vi "SET_ToolGraphic.vi"(8 "error in":errorcluster, 9 "Temp Coord":T5, 10 "Temp Icon":picture, 11 "Data in":T1={"Class"={"Ants"=refnum, "Layer"=refnum, "Templates"=refnum, "Icon"=refnum, "Glyph"=refnum, "Settings"=refnum, "Tools"=refnum, "History"=refnum}, "Ref"={"Add Layer"=refnum, "Remove Layer"=refnum, "Line Text"=[], "Body Text Spec"=refnum, "DNL_Font"=refnum, "glyph path str"=refnum, "templates path str"=refnum, "Arrow Up"=refnum, "Arrow Down"=refnum, "IE VI Ref"=refnum, "Glyphs tree"=refnum, "Templates tree"=refnum, "Layer Icon Text"=refnum, "Layer Template"=refnum, "Body Text"=refnum, "Search Templates"=refnum, "TextMarker"=refnum, "Tab Control"=refnum, "Search Glyphs"=refnum, "Line Color"=refnum, "DNL_Glyphs []"=refnum, "Fill Color"=refnum, "Tools"=refnum, "Icon"=refnum, "Preview"=refnum, "Ants"=refnum, "Terminals"=refnum, "menu reference"=refnum, "LayerNames"=[], "GlyphLoadAnimation"=refnum, "TemplateLoadAnimation"=refnum, "refreshGlyphs"=refnum, "refreshTemplates"=refnum}, "Support"={"AntsRect"={"left"=0, "top"=0, "right"=0, "bottom"=0}, "Mouse Move Coords"={"Horizontal"=0, "Vertical"=0}, "Mouse Down Coords"={"Horizontal"=0, "Vertical"=0}, "Temp Coord"={"Horizontal"=0, "Vertical"=0}, "Action"=enum."Default", "Edge Color"=4914962, "Fill Color"=16860, "Mouse Down?"=FALSE, "Draft Mode?"=FALSE, "Temp Icon"=bytes[3102], "CTRL Pressed"=FALSE, "Move Selection?"=FALSE, "AntsRect Orig"={"left"=0, "top"=0, "right"=0, "bottom"=0}, "Text"="", "TM Set?"=FALSE, "Mouse inside icon?"=FALSE, "Tool (old value)"=0, "Pencil Move Color"=0, "Swap Colors?"=FALSE, "Shift pressed?"=FALSE}}) -> (0 "error out":errorcluster, 1 "All Layers":refnum<class "Layer.lvclass">[](array[class]), 3 "Data out":T1={"Class"={"Ants"=refnum, "Layer"=refnum, "Templates"=refnum, "Icon"=refnum, "Glyph"=refnum, "Settings"=refnum, "Tools"=refnum, "History"=refnum}, "Ref"={"Add Layer"=refnum, "Remove Layer"=refnum, "Line Text"=[], "Body Text Spec"=refnum, "DNL_Font"=refnum, "glyph path str"=refnum, "templates path str"=refnum, "Arrow Up"=refnum, "Arrow Down"=refnum, "IE VI Ref"=refnum, "Glyphs tree"=refnum, "Templates tree"=refnum, "Layer Icon Text"=refnum, "Layer Template"=refnum, "Body Text"=refnum, "Search Templates"=refnum, "TextMarker"=refnum, "Tab Control"=refnum, "Search Glyphs"=refnum, "Line Color"=refnum, "DNL_Glyphs []"=refnum, "Fill Color"=refnum, "Tools"=refnum, "Icon"=refnum, "Preview"=refnum, "Ants"=refnum, "Terminals"=refnum, "menu reference"=refnum, "LayerNames"=[], "GlyphLoadAnimation"=refnum, "TemplateLoadAnimation"=refnum, "refreshGlyphs"=refnum, "refreshTemplates"=refnum}, "Support"={"AntsRect"={"left"=0, "top"=0, "right"=0, "bottom"=0}, "Mouse Move Coords"={"Horizontal"=0, "Vertical"=0}, "Mouse Down Coords"={"Horizontal"=0, "Vertical"=0}, "Temp Coord"={"Horizontal"=0, "Vertical"=0}, "Action"=enum."Default", "Edge Color"=4914962, "Fill Color"=16860, "Mouse Down?"=FALSE, "Draft Mode?"=FALSE, "Temp Icon"=bytes[3102], "CTRL Pressed"=FALSE, "Move Selection?"=FALSE, "AntsRect Orig"={"left"=0, "top"=0, "right"=0, "bottom"=0}, "Text"="", "TM Set?"=FALSE, "Mouse inside icon?"=FALSE, "Tool (old value)"=0, "Pencil Move Color"=0, "Swap Colors?"=FALSE, "Shift pressed?"=FALSE}})   [LabVIEW 2020]
uses:
  vi.lib/LabVIEW Icon API/lv_icon/Classes/Layer/Layer.lvclass
  Class/Ants/Ants.lvclass
  Class/FakedArray/FakedArray.lvclass
  vi.lib/LabVIEW Icon API/lv_icon/Classes/Icon/Icon.lvclass
  Class/Icon Library/Glyph.lvclass
  Class/Settings/Settings.lvclass
  Class/Tools/Tools Paint.lvclass
  vi.lib/LabVIEW Icon API/lv_icon/Controls/LayerType.ctl
  <vilib>/Utility/miscctls.llb/LVPoint32TypeDef.ctl
  Controls/SupportClass_Action.ctl
  vi.lib/LabVIEW Icon API/lv_icon/Controls/IEColor.ctl
  Controls/Support Cluster.ctl
  lv_icon.lvlib
  Controls/References Cluster.ctl
  Controls/IE Classes.ctl
  Controls/Global Data.ctl
  History/History/History.lvclass
panel:
  in  "FileName":string="Tool"
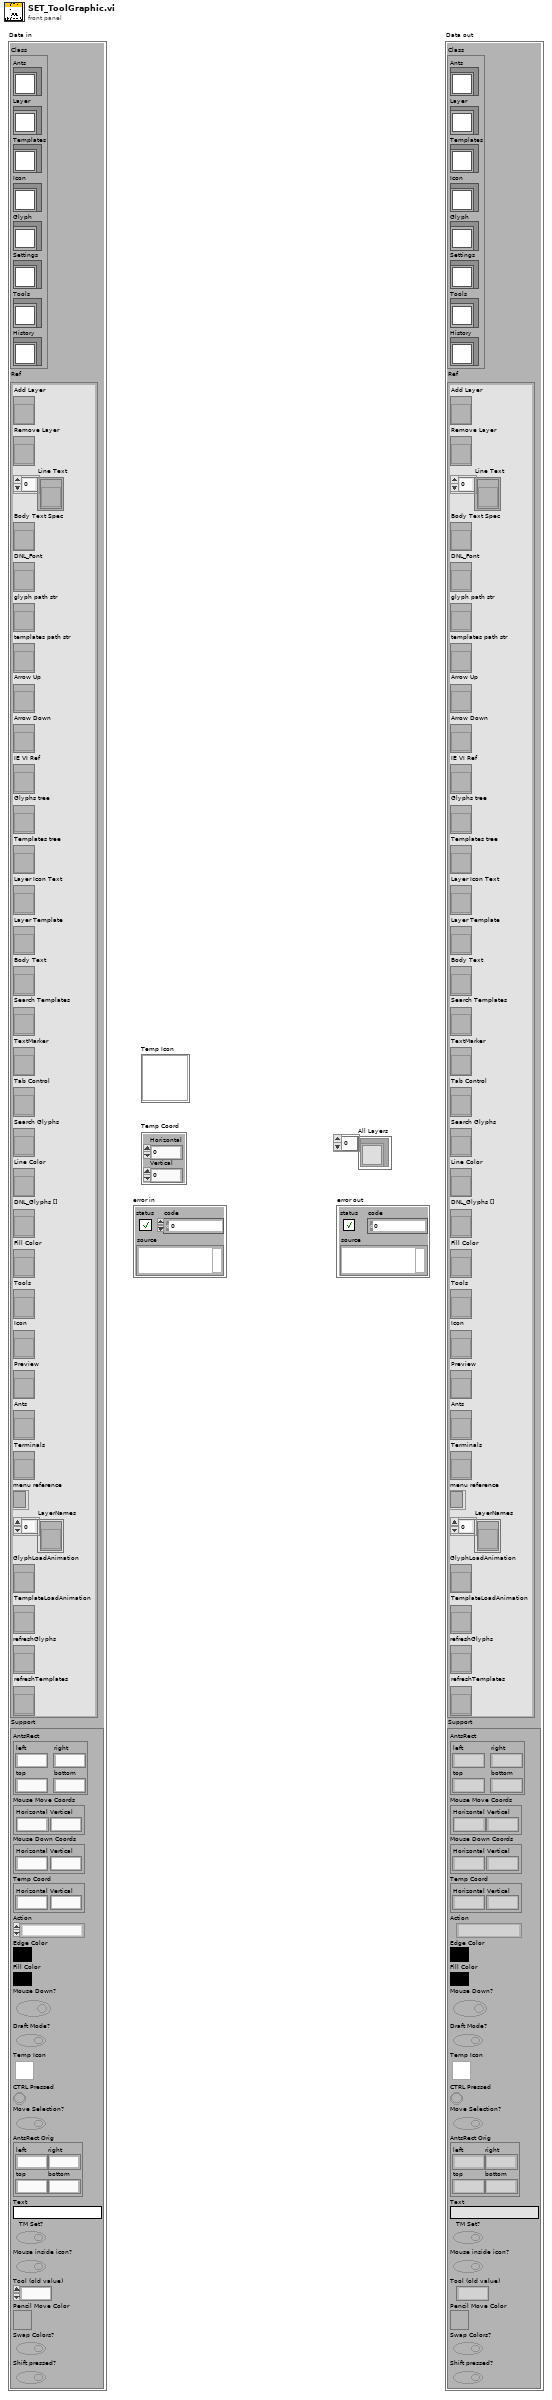
[diagram p1: front panel]
types:
  T1 = typedef "lv_icon.lvlib/Global Data.ctl" = cluster{"Class":T2, "Ref":T3, "Support":T4}
  T2 = typedef "lv_icon.lvlib/IE Classes.ctl" = cluster{"Ants":refnum<class "Ants.lvclass">, "Layer":refnum<class "FakedArray.lvclass">, "Templates":refnum<class "FakedArray.lvclass">, "Icon":refnum<class "Icon.lvclass">, "Glyph":refnum<class "Glyph.lvclass">, "Settings":refnum<class "Settings.lvclass">, "Tools":refnum<class "Tools Paint.lvclass">, "History":refnum<class "History.lvclass">}
  T3 = typedef "lv_icon.lvlib/References Cluster.ctl" = cluster{"Add Layer":refnum<vi>, "Remove Layer":refnum<vi>, "Line Text":refnum<vi>[], "Body Text Spec":refnum<vi>, "DNL_Font":refnum<vi>, "glyph path str":refnum<vi>, "templates path str":refnum<vi>, "Arrow Up":refnum<vi>, "Arrow Down":refnum<vi>, "IE VI Ref":refnum<vi>, "Glyphs tree":refnum<vi>, "Templates tree":refnum<vi>, "Layer Icon Text":refnum<vi>, "Layer Template":refnum<vi>, "Body Text":refnum<vi>, "Search Templates":refnum<vi>, "TextMarker":refnum<vi>, "Tab Control":refnum<vi>, "Search Glyphs":refnum<vi>, "Line Color":refnum<vi>, "DNL_Glyphs []":refnum<vi>, "Fill Color":refnum<vi>, "Tools":refnum<vi>, "Icon":refnum<vi>, "Preview":refnum<vi>, "Ants":refnum<vi>, "Terminals":refnum<vi>, "menu reference":refnum<k9>, "LayerNames":refnum<vi>[], "GlyphLoadAnimation":refnum<vi>, "TemplateLoadAnimation":refnum<vi>, "refreshGlyphs":refnum<vi>, "refreshTemplates":refnum<vi>}
  T4 = typedef "lv_icon.lvlib/Support Cluster.ctl" = cluster{"AntsRect":cluster{"left":i16, "top":i16, "right":i16, "bottom":i16}, "Mouse Move Coords":T5, "Mouse Down Coords":T5, "Temp Coord":T5, "Action":T6, "Edge Color":T7, "Fill Color":T7, "Mouse Down?":bool, "Draft Mode?":bool, "Temp Icon":picture, "CTRL Pressed":bool, "Move Selection?":bool, "AntsRect Orig":cluster{"left":i16, "top":i16, "right":i16, "bottom":i16}, "Text":string, "TM Set?":bool, "Mouse inside icon?":bool, "Tool (old value)":u32, "Pencil Move Color":u32, "Swap Colors?":bool, "Shift pressed?":bool}
  T5 = typedef "LVPoint32TypeDef.ctl" = cluster{"Horizontal":i32, "Vertical":i32}
  T6 = typedef "SupportClass_Action.ctl" = enum16{"Default", "Move Selection", "Glyph Library", "Tool"}
  T7 = typedef "IEColor.ctl" = u32
  T8 = cluster{"left":i16, "top":i16, "right":i16, "bottom":i16}
  T9 = typedef "lv_icon.lvlib/INI Data.ctl" = cluster{"Show Terminals?":bool, "Text":cluster{"Font":T10, "Alignment":T11, "Size":T12}, "3rd party Templates":cluster{"Store 3rd party Templates?":bool, "Folder Name":string}, "Merge user layers on commit":bool, "Body Text":T13, "Fill Color":T7, "Edge Color":T7, "Tab":u16, "Tool":T14, "Disable Layers?":bool}
  T10 = typedef "Font.ctl" = string
  T11 = typedef "Alignment.ctl" = u16
  T12 = typedef "Font Size.ctl" = u8
  T13 = typedef "BodyText.ctl" = cluster{"Line 1 text":string, "Line 2 text":string, "Line 3 text":string, "Line 4 text":string, "Line 1 color":u32, "Line 2 color":u32, "Line 3 color":u32, "Line 4 color":u32, "Body Text Spec":cluster{"Font":T10, "Alignment":T11, "Size":u8}, "Center text vertically":bool, "Capitalize Text":bool}
  T14 = typedef "Tools.ctl" = enum32{"Pencil", "Line", "Dropper", "Fill", "Rectangle", "Filled Rectangle", "Ellipse", "Filled Ellipse", "Eraser", "Text", "Select", "Move"}
  T15 = typedef "LayerType.ctl" = enum16{"Graphic", "Text", "Tool", "Graphic Drop"}
  T16 = typedef "Layer.ctl" = cluster{"LayerIcon":picture, "LayerName":string, "Opacity":u8, "Visibility?":bool}
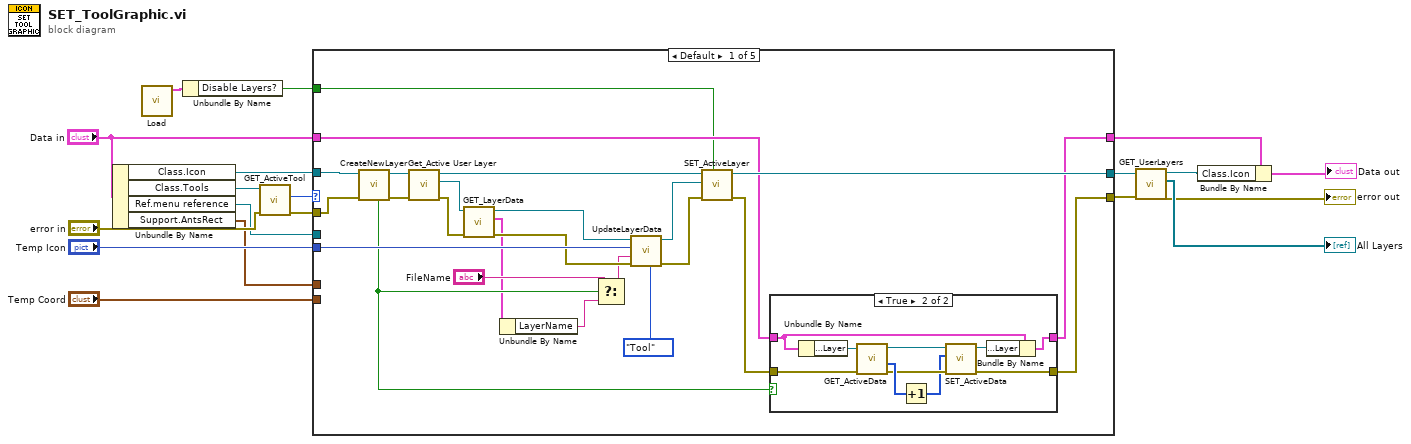
[diagram p0: block diagram]
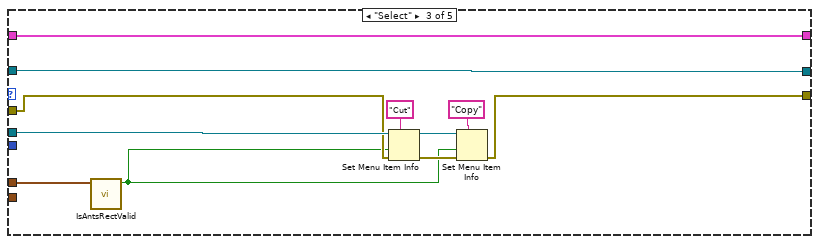
[diagram p4: hidden frame]
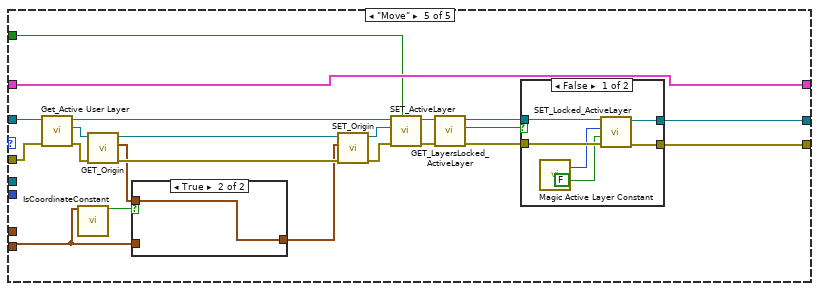
[diagram p6: hidden frame]
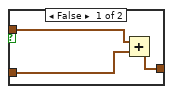
[diagram p8: hidden frame]
diagram:
  n1 = Unbundle By Name("Data in") -> ("Class.Icon"=w11:refnum<class "Icon.lvclass">, "Class.Tools"=w12:refnum<class "Tools Paint.lvclass">, "Ref.menu reference"=w4:refnum<k9>, "Support.AntsRect"=w3:T8)
  n2 = call "Load.vi"() -> ("INI Data"=w2:T9)  [unwired: 3 in, 8 out]
  n3 = Unbundle By Name(w2) -> ("Disable Layers?"=w1:bool)
  n4 = call-dynamic "GET_ActiveTool.vi"("error in (no error)"="error in", "Tools Paint.lvclass in"=w12) -> ("error out"=w14:errorcluster, "Radio Buttons"=w13:T14)  [unwired: 8 out]
  n5 = case shown="Default" w13 {
    tunnel: w11 -> [w43 w58 w69 w72 w93]
    tunnel: "Temp Icon" -> [w37 _ _ _ _]
    tunnel: [w36 w58 w69 w72 w77] -> w18
    tunnel: [w21 w57 w61 w71 w76] -> w19
    tunnel: "Temp Coord" -> [_ _ _ _ w84]
    tunnel: w14 -> [w34 w57 w62 w71 w75]
    tunnel: "Data in" -> [w23 w56 w68 w70 w74]
    tunnel: [w22 w56 w68 w70 w74] -> w8
    tunnel: w4 -> [_ _ w63 _ _]
    tunnel: w3 -> [_ _ w60 _ _]
    tunnel: w1 -> [w20 _ _ _ w73]
    frame Default {
      n6 = call "CreateNewLayer.vi"("error in"=w34, "Icon.lvclass"=w43) -> ("error out"=w41:errorcluster, "Icon.lvclass out"=w42:refnum<class "Icon.lvclass">, "Layer added?"=w32:bool)  [unwired: 3 in, 4 out]
      n7 = call-dynamic "Get_Active User Layer.vi"("error in (no error)"=w41, "Icon in"=w42) -> ("error out"=w30:errorcluster, "Layer.lvclass"=w28:refnum<class "Layer.lvclass">, "Icon out"=w40:refnum<class "Icon.lvclass">)  [unwired: 7 out]
      n8 = call-dynamic "GET_LayerData.vi"("error in (no error)"=w30, "Layer.lvclass in"=w28) -> ("error out"=w29:errorcluster, "Data"=w26:T16, "Layer.lvclass out"=w27:refnum<class "Layer.lvclass">)  [unwired: 7 out]
      n9 = Unbundle By Name(w26) -> ("LayerName"=w25:string)
      n10 = Select(t="FileName", s=w32, f=w25) -> (s? t:f=w24:string)
      n11 = call "UpdateLayerData.vi"("Type"=LayerType."Tool", "error in"=w29, "LayerName"=w24, "new picture"=w37, "Active Layer"=w27) -> ("error out"=w38:errorcluster, "Layer.lvclass out"=w39:refnum<class "Layer.lvclass">)  [unwired: 3 in, 2 out]
      n12 = call-dynamic "SET_ActiveLayer.vi"("Combine User Layers?"=w20, "error in (no error)"=w38, "Layer.lvclass"=w39, "Icon.lvclass in"=w40) -> ("error out"=w33:errorcluster, "Icon.lvclass out"=w36:refnum<class "Icon.lvclass">)  [unwired: 6 out]
      n13 = case shown="True" w32 {
        tunnel: w33 -> [w45 w46]
        tunnel: [w45 w48] -> w21
        tunnel: w23 -> [w44 w50]
        tunnel: [w44 w47] -> w22
        frame False {
        }
        frame True {
          n14 = Unbundle By Name(w50) -> ("Class.Layer"=w51:refnum<class "FakedArray.lvclass">)
          n15 = call-dynamic "GET_ActiveData.vi"("error in (no error)"=w46, "FakedArray in"=w51) -> ("error out"=w53:errorcluster, "Active Data []"=w54:i32[], "FakedArray out"=w55:refnum<class "FakedArray.lvclass">)  [unwired: 7 out]
          n16 = Increment(x=w54) -> (x+1=w52:i32[])
          n17 = call-dynamic "SET_ActiveData.vi"("error in (no error)"=w53, "Active Data"=w52, "FakedArray.lvclass in"=w55) -> ("error out"=w48:errorcluster, "FakedArray.lvclass out"=w49:refnum<class "FakedArray.lvclass">)  [unwired: 7 out]
          n18 = Bundle By Name(cluster=w50, "Class.Layer"=w49) -> (w47:T1)
        }
      }
    }
    frame "Fill" {
    }
    frame "Select" {
      n19 = call "IsAntsRectValid.vi"("AntsRect"=w60) -> ("Valid?"=w59:bool)  [unwired: 10 out]
      n20 = Set Menu Item Info(7:"Cut" ("item tag"), 8:w62, 9:w59, 11:w63) -> (0:w67:errorcluster, 3:w65:refnum<k9>)  [unwired: 3 out]
      n21 = Set Menu Item Info(7:"Copy" ("item tag"), 8:w67, 9:w59, 11:w65) -> (0:w61:errorcluster)  [unwired: 4 out]
    }
    frame "Dropper", "Eraser" {
    }
    frame "Move" {
      n22 = call-dynamic "Get_Active User Layer.vi"("error in (no error)"=w75, "Icon in"=w93) -> ("error out"=w88:errorcluster, "Layer.lvclass"=w90:refnum<class "Layer.lvclass">, "Icon out"=w94:refnum<class "Icon.lvclass">)  [unwired: 7 out]
      n23 = call "IsCoordinateConstant.vi"("Coordinate"=w84) -> ("Constant?"=w83:bool)  [unwired: 10 out]
      n24 = call-dynamic "GET_Origin.vi"("error in (no error)"=w88, "Layer.lvclass in"=w90) -> ("error out"=w87:errorcluster, "Point32"=w86:T5, "Layer.lvclass out"=w89:refnum<class "Layer.lvclass">)  [unwired: 7 out]
      n25 = case shown="True" w83 {
        tunnel: w86 -> [w105 w106]
        tunnel: [w103 w106] -> w85
        tunnel: w84 -> [w104 _]
        frame False {
          n26 = Add(x=w105, y=w104) -> (x+y=w103:T5)
        }
        frame True {
        }
      }
      n27 = call-dynamic "SET_Origin.vi"("error in"=w87, "Point32"=w85, "Layer.lvclass in"=w89) -> ("error out"=w91:errorcluster, "Layer.lvclass out"=w92:refnum<class "Layer.lvclass">)  [unwired: 7 out]
      n28 = call-dynamic "SET_ActiveLayer.vi"("Combine User Layers?"=w73, "error in (no error)"=w91, "Layer.lvclass"=w92, "Icon.lvclass in"=w94) -> ("error out"=w82:errorcluster, "Icon.lvclass out"=w81:refnum<class "Icon.lvclass">)  [unwired: 6 out]
      n29 = call-dynamic "GET_LayersLocked_ActiveLayer.vi"("error in (no error)"=w82, "Icon.lvclass in"=w81) -> ("error out"=w78:errorcluster, "Layers Locked?"=w80:bool, "Icon.lvclass out"=w79:refnum<class "Icon.lvclass">)  [unwired: 7 out]
      n30 = case shown="False" w80 {
        tunnel: w79 -> [w100 w102]
        tunnel: w78 -> [w99 w101]
        tunnel: [w97 w102] -> w77
        tunnel: [w96 w101] -> w76
        frame False {
          n31 = call "Magic Active Layer Constant.vi"() -> ("Magic Constant"=w95:i32)  [unwired: 19 out]
          n32 = call-dynamic "SET_Locked_ActiveLayer.vi"("error in (no error)"=w99, "Layers Locked?"=FALSE, "Active Layer"=w95, "Icon.lvclass in"=w100) -> ("error out"=w96:errorcluster, "Icon.lvclass out"=w97:refnum<class "Icon.lvclass">)  [unwired: 6 out]
        }
        frame True {
        }
      }
    }
  }
  n33 = call-dynamic "GET_UserLayers.vi"("error in (no error)"=w19, "Icon.lvclass in"=w18) -> ("error out"=→"error out":errorcluster, "All Layers"=→"All Layers":refnum<class "Layer.lvclass">[], "Icon.lvclass out"=w7:refnum<class "Icon.lvclass">)  [unwired: 7 out]
  n34 = Bundle By Name(cluster=w8, "Class.Icon"=w7) -> (→"Data out":T1)
